vi "Get Channel Name.vi"(0 "measurement context in":refnum<class "Measure Call Context.lvclass">, 5 "Pin Name[]":string[](array[string]), 11 "error in (no error)":errorcluster) -> (4 "Channel Name":string[](array[string]), 6 "Channel Number":string[](array[string]), 8 "Session Exists":bool[](array[boolean]), 10 "Session.name":string[](array[string]), 15 "error out":errorcluster)   [LabVIEW 2024, in "devicePowerSequencerCoreLogic.lvlib"]
uses:
  devicePowerSequencerCoreLogic.lvlib
  <vilib>/Plug-In SDKs/Measurements/Measure Call Context/Measure Call Context.lvclass
  <vilib>/Plug-In SDKs/Sessions/niDCPower/NI Session Management niDCPower.lvlib
  <vilib>/Plug-In SDKs/Clients/Session Management V1/Session Reservation/Session Reservation.lvclass
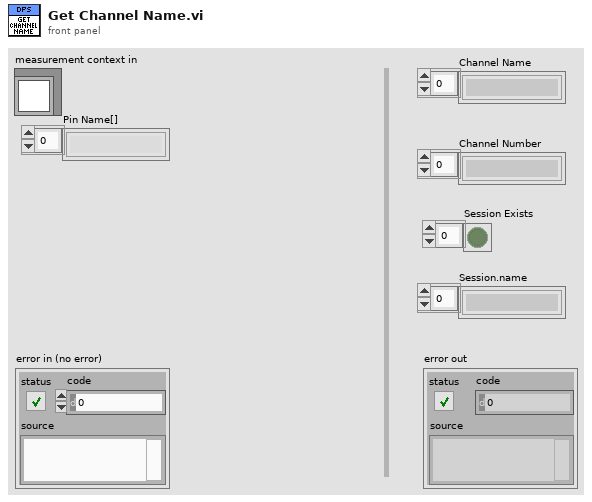
[diagram p1: front panel]
types:
  T1 = typedef "NI Session Management niDCPower.lvlib/Connection with Session.ctl" = cluster{"connection":T2, "session":refnum<k15>}
  T2 = typedef "NI Session Management V1 Client.lvlib/Session Reservation.lvclass/Connection.ctl" = cluster{"pin or relay name":string, "site":i32, "instrument type id":string, "channel":string}
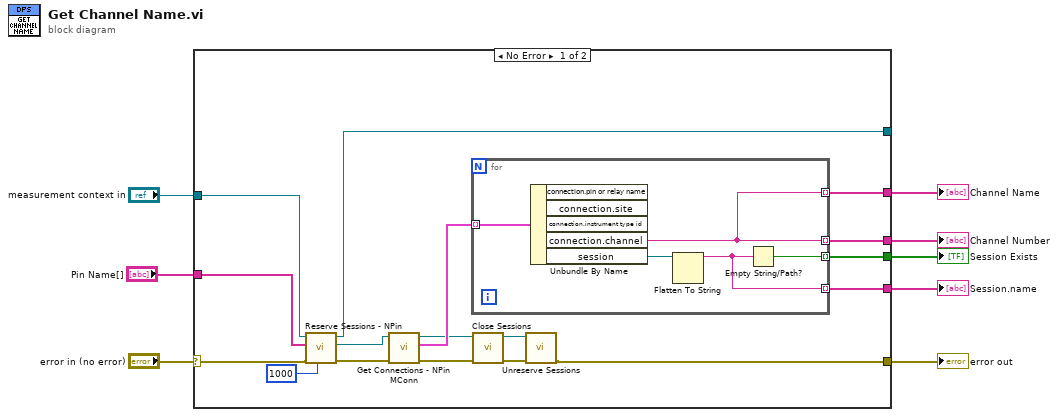
[diagram p0: block diagram]
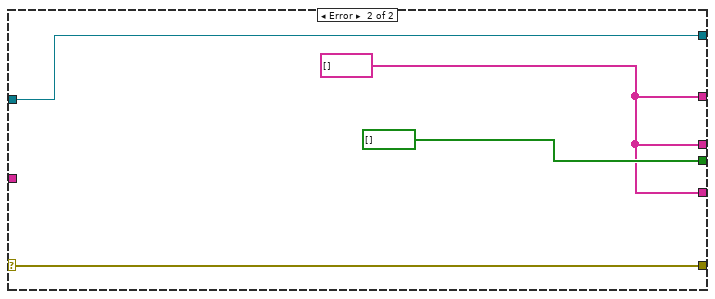
[diagram p2: hidden frame]
diagram:
  n1 = case shown="No Error" "error in (no error)" {
    selector: "error in (no error)" -> [w17 w34]
    tunnel: "Pin Name[]" -> [w16 _]
    tunnel: [w18 w34] -> w6
    tunnel: [w15 w32] -> w5
    tunnel: [w14 w32] -> w4
    tunnel: [w12 w32] -> w3
    tunnel: [w13 bool[] []] -> w2
    tunnel: "measurement context in" -> [w11 w31]
    tunnel: [w9 w31] -> _
    frame No Error {
      n2 = call <vilib>:"Reserve Sessions - NPin.vi"("timeout (ms)"=1000, "error in"=w17, "pin or relay names"=w16, "measurement context in"=w11) -> ("error out"=w21:errorcluster, "session reservation out"=w24:refnum<class "Session Reservation.lvclass">, "measurement context out"=w9:refnum<class "Measure Call Context.lvclass">)  [unwired: 5 in]
      n3 = call <vilib>:"Get Connections - NPin MConn.vi"("error in"=w21, "session reservation in"=w24) -> ("error out"=w22:errorcluster, "connections"=w25:T1[], "session reservation out"=w23:refnum<class "Session Reservation.lvclass">)  [unwired: 7 in]
      n4 = for {
        tunnel: w25 -> [w30] mode=indexing
        tunnel: [w28] -> w12 mode=indexing
        tunnel: [w27] -> w13 mode=indexing
        tunnel: [w26] -> w14 mode=indexing
        tunnel: [w26] -> w15 mode=indexing
        n5 = Unbundle By Name(w30) -> ("connection.channel"=w26:string, "session"=w29:refnum<k15>)  [unwired: 3 out]
        n6 = Flatten To String(anything=w29) -> (data string=w28:string)  [unwired: 3 in, 2 out]
        n7 = Empty String/Path?(string/path=w28) -> (empty?=w27:bool)
      }
      n8 = call <vilib>:"Close Sessions.vi"("error in"=w22, "session reservation in"=w23) -> ("error out"=w20:errorcluster, "session reservation out"=w19:refnum<class "Session Reservation.lvclass">)  [unwired: 8 in]
      n9 = call <vilib>:"Unreserve Sessions.vi"("error in"=w20, "session reservation in"=w19) -> ("error out"=w18:errorcluster)  [unwired: 9 in]
    }
    frame Error {
      w32 = string[] []
    }
  }
  "error out" <- w6
  "Channel Name" <- w5
  "Channel Number" <- w4
  "Session Exists" <- w2
  "Session.name" <- w3
